vi "editDialog.vi"(0 "reference":refnum<class "StateTransitionEdge.lvclass">, 5 "error in (no error)":errorcluster) -> (14 "reference out":refnum<class "StateTransitionEdge.lvclass">, 15 "cancel":bool, 19 "error out":errorcluster)   [LabVIEW 2020, in "StateTransitionEdge.lvclass"]
doc: "Edit Dialog"
uses:
  <resource>/Framework/Providers/Open_GDS/UML/StateTransitionEdge_class/StateTransitionEdge.lvclass
  C:/Program Files (x86)/National Instruments/LabVIEW 2020/resource/Framework/Providers/Open_GDS/UML/ClassRelationshipEdge_class/ClassRelationshipEdge.lvclass
  C:/Program Files (x86)/National Instruments/LabVIEW 2020/resource/Framework/Providers/Open_GDS/UML/SegmentedLineEdge_class/SegmentedLineEdge.lvclass
  <resource>/Framework/Providers/Open_GDS/UML/BentStyle_class/BentStyleType.ctl
  <resource>/Framework/Providers/Open_GDS/UML/ContextHelp/ContextHelp_HelpTexts.ctl
  <resource>/Framework/Providers/Open_GDS/UML/BentStyle_class/BentStyle.lvclass
  <resource>/Framework/Providers/Open_GDS/UML/ClassRelationshipEdge_class/ClassRelationshipEdge.lvclass
  <resource>/Framework/Providers/Open_GDS/UML/SegmentedLineEdge_class/SegmentedLineEdge.lvclass
panel:
  in  "Bent Style":T1
  in  "Help":bool
  in  "Event":string
  in  "Cancel Button":bool
  in  "OK Button":bool
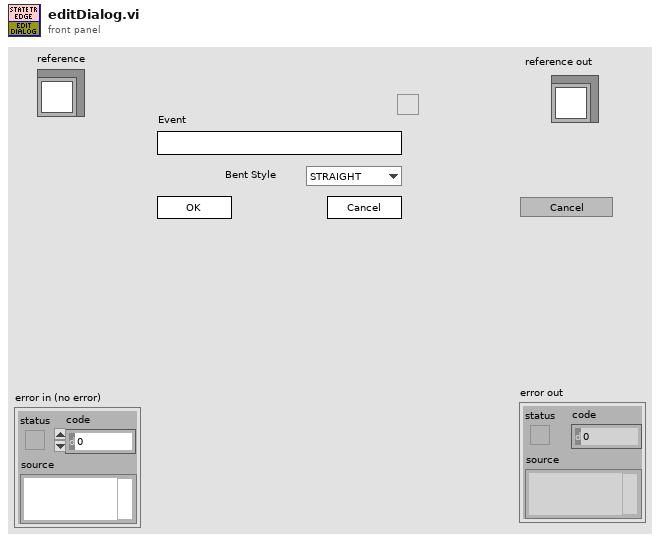
[diagram p1: front panel]
types:
  T1 = typedef "BentStyle.lvclass/BentStyleType.ctl" = enum16{"STRAIGHT", "HV", "VH", "HVH", "VHV", "ARC"}
  T2 = typedef "ContextHelp_HelpTexts.ctl" = enum16{"None(Hide)", "Default", "Help", "Welcome", "GettingStarted", "ClassDiagram_Help", "SequenceDiagram_Help", "UseCaseDiagram_Help", "BSelect", "BClass", "BInterface", "BPackage", "BNote", "BDependency", "BInheritance", "BInterfaceImplementation", "BAssociation", "BAggregation", "BCompAggregation", "BNoteConnector", "BObject", "BActionBar", "BCall", "BSystem", "BActor", "BUseCase", "BGeneralization", "BIncludes", "BExtends", "BUseCaseDiagramAssociation", "ClassRelationshipEdge editDialog_Bent Style", "ClassRelationshipEdge editDialog_RelationType", "ClassRelationshipEdge editDialog_Reverse association", "ClassRelationshipEdge editDialog_Start label", "ClassRelationshipEdge editDialog_Middle label", "ClassRelationshipEdge editDialog_End label", "UMLEditor reversedEngineering_Pathes", "ReversedEngineering StateReverseDialog_Help", "ReversedEngineering StateQueuedSettings_Help", "UMLEditor reversedEngineering_AddTopVIs", "UMLEditor reversedEngineering_AddClasses", "UMLEditor reversedEngineering_AddDirs", "UMLEditor reversedEngineering_Recursively", "UMLEditor reversedEngineering_Remove", "UMLEditor reversedEngineering_ClearList", "UMLEditor reversedEngineering_HideSubAss", "UMLEditor reversedEngineering_CreateTypes", "UMLEditor reversedEngineering_OnlyInheritance", "UMLEditor reversedEngineering_CreateApplication", "UMLEditor reversedEngineering_OK", "UMLEditor reversedEngineering_Cancel", "UMLEditor reversedEngineering_Help", "UMLEditor createWizardScriptFile_ScriptfilePath", "UMLEditor createWizardScriptFile_ClassPath", "UMLEditor createWizardScriptFile_Use", "UMLEditor createWizardScriptFile_PrivateDirName", "UMLEditor createWizardScriptFile_DirAppend", "UMLEditor createWizardScriptFile_Separator Character", "UMLEditor createWizardScriptFile_OK", "UMLEditor createWizardScriptFile_Cancel", "UMLEditor createWizardScriptFile_Help", "ClassNode editDialog_Class Name", "InterfaceNode editDialog_Class Name", "ClassNode editDialog_Attribute", "ClassNode editDialog_Methods", "InterfaceNode editDialog_Methods", "ClassNode editDialog_connection", "InterfaceNode editDialog_connection", "ClassNode editDialog_StereoType", "ClassNode editDialog_ShowAttrib", "ClassNode editDialog_ShowMethods", "ClassNode editDialog_ClassPath", "ClassNode editDialog_AddAttribute", "ClassNode editDialog_AddMethod", "InterfaceNode editDialog_AddMethod", "ClassNode AttributeGuide_AttributeName", "ClassNode AttributeGuide_Array?", "ClassNode AttributeGuide_Data Type", "ClassNode AttributeGuide_RefName", "ClassNode AttributeGuide_Preview", "ClassNode AttributeGuide_OK", "ClassNode AttributeGuide_Cancel", "ClassNode MethodGuide_Visibility", "ClassNode MethodGuide_Method Name", "ClassNode MethodGuide_Preview", "ClassNode MethodGuide_OK", "ClassNode MethodGuide_Cancel", "CallNode EditCallProperties_AllButtons", "ObjectNode EditObjectlProperties_AllButtons", "ActorNode EditActorProperties_AllButtons", "UseCaseRelationshipNode EditUseCaselProperties_AllButtons", "UseCaseNode EditUseCaselProperties_AllButtons", "SystemNode EditSystemProperties_AllButtons", "ReversedEngineering UpdateAttributes_AllButtons", "StateNode editDialog_AllButtons", "StateTransition editDialog_AllButtons", "ArrangeNodes Main_Picture", "ArrangeNodes Main_Zoom", "ArrangeNodes Main_Auto Zoom", "ArrangeNodes Main_shorten", "ArrangeNodes Main_Min Length", "ArrangeNodes Main_Max Length", "ArrangeNodes Main_increase", "ArrangeNodes Main_decrease", "ArrangeNodes Main_Shake", "ArrangeNodes Main", "BState", "BInitialState", "BFinalState", "BStateTransition", "StateDiagram_Help", "StateDiagram_PropertiesAllButtons", "ReversedEngineering StateReverseDialog_ClearStates", "ReversedEngineering StateReverseDialog_UseQueuedStateMachines", "ReversedEngineering StateReverseDialog_QueuedSettings", "ReversedEngineering StateReverseDialog_SearchForVIs", "ReversedEngineering StateReverseDialog_SearchCriteria", "OptionsDialog_ClassBasePath", "OptionsDialog_VIPath", "OptionsDialog_ApplicationPath", "OptionsDialog_WizDir", "OptionsDialog_IniFilePath", "OptionsDialog_DefineColors", "OptionsDialog_Help", "OptionsDialog_CreateTypes", "ClassRelationshipEdge editDialog_SplitWire"}
  T3 = typedef "ClassRelationshipEdge.lvclass/ObjectAttributes.ctl" = cluster{"bentStyleRef":refnum<class "BentStyle.lvclass">, "startConnectionOffset":cluster{"x":i32, "y":i32}, "endConnectionOffset":cluster{"x":i32, "y":i32}, "MidLineOffset":cluster{"x":i32, "y":i32}, "DepClass":T4}
  T4 = typedef "ReversedEngineering_ViDependencyDetailsType.ctl" = cluster{"ThisVIs/Ctls":path[], "Dependent_VIs/Ctls":path[]}
  T5 = typedef "SegmentedLineEdge.lvclass/ObjectAttributes.ctl" = cluster{"lineStyle":refnum<class "LineStyle.lvclass">, "startArrowHead":refnum<class "ArrowHead.lvclass">, "endArrowHead":refnum<class "ArrowHead.lvclass">, "startLabel":string, "midLabel":string, "endLabel":string, "MidLabelOffset":T6, "SplitWire":bool}
  T6 = typedef "Point Point2D.ctl" = cluster{"x":dbl, "y":dbl}
  T7 = typedef "ContextHelp_ShowType.ctl" = cluster{"Header":string, "Picture":picture, "Text":string}
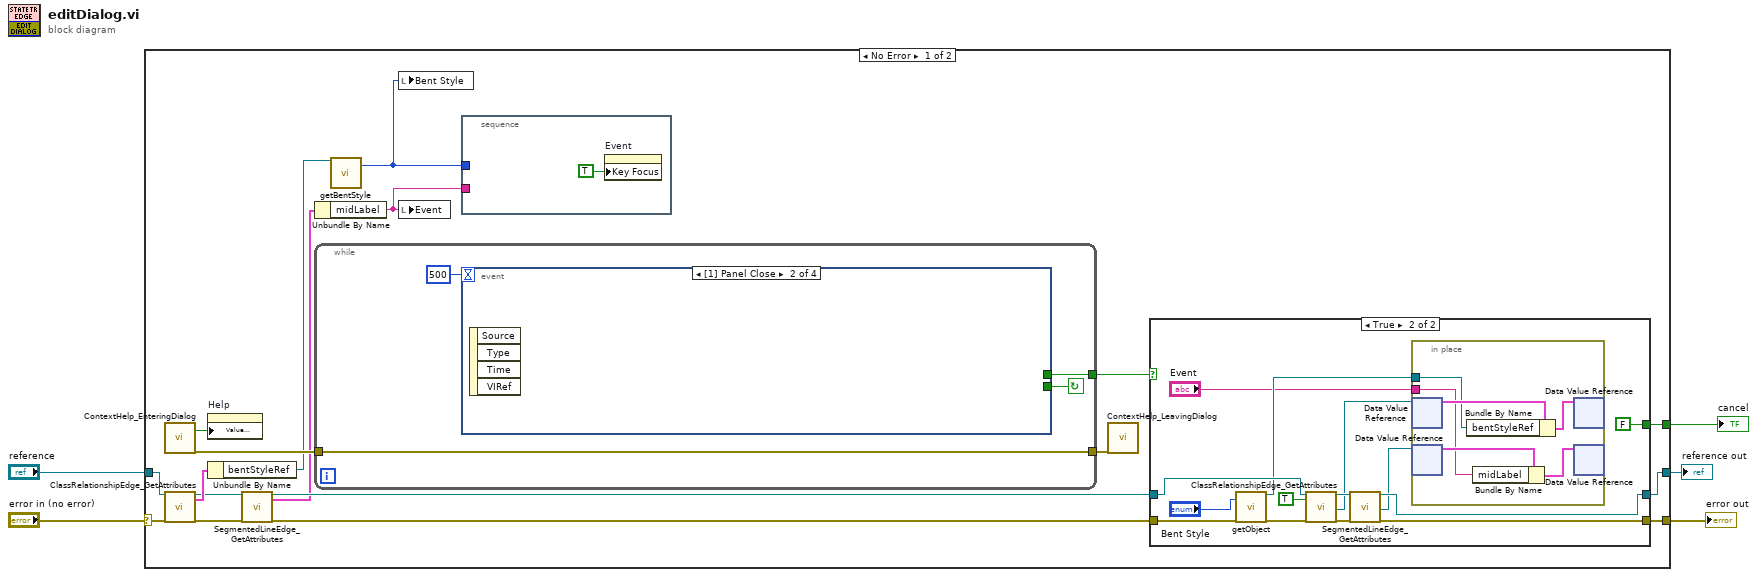
[diagram p0: block diagram]
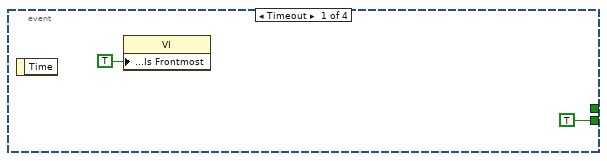
[diagram p2: hidden frame]
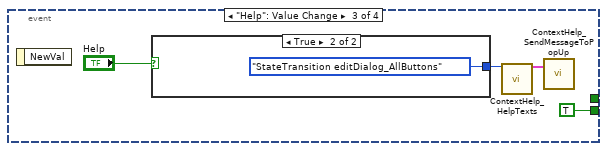
[diagram p3: hidden frame]
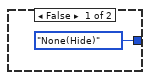
[diagram p4: hidden frame]
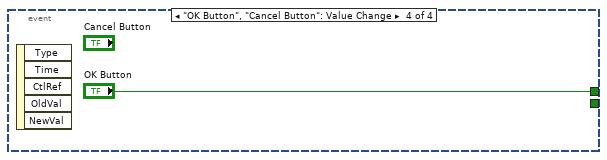
[diagram p5: hidden frame]
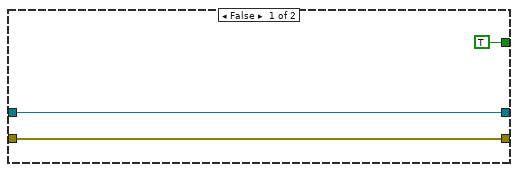
[diagram p6: hidden frame]
diagram:
  n1 = case shown="No Error" "error in (no error)" {
    selector: "error in (no error)" -> [w20 w61]
    tunnel: "reference" -> [w21 w62]
    tunnel: [w23 w61] -> w3
    tunnel: [w22 w62] -> w2
    tunnel: [w17 _] -> w1
    frame No Error {
      n2 = call <resource>:"ContextHelp_EnteringDialog.vi"() -> ("HelpStatus"=w16:bool, "error out"=w14:errorcluster)  [unwired: 3 in, 15 out]
      n3 = call <resource>:"ClassRelationshipEdge_GetAttributes.vi"("reference in"=w21, "error in (no error)"=w20) -> ("reference out"=w10:refnum<class "StateTransitionEdge.lvclass">, "Data"=w11:T3, "error out"=w9:errorcluster)  [unwired: 14 in, 1 out]
      n4 = property on="Help" class="Bool (strict)"("Value (Signaling)"=w16) -> ()  [unwired: 2 in, 2 out]
      n5 = Unbundle By Name(w11) -> ("bentStyleRef"=w13:refnum<class "BentStyle.lvclass">)
      n6 = call <resource>:"SegmentedLineEdge_GetAttributes.vi"("reference in"=w10, "error in (no error)"=w9) -> ("reference out"=w7:refnum<class "StateTransitionEdge.lvclass">, "Data"=w6:T5, "error out"=w8:errorcluster)  [unwired: 14 in, 1 out]
      n7 = Unbundle By Name(w6) -> ("midLabel"=w18:string)
      n8 = while {
        tunnel: [w27] -> w19
        tunnel: [w24] -> w15
        tunnel: w14 -> [w24]
        stop <- w26 continue-if-true
        n9 = event shown="[1] Panel Close" {
          selector: _ -> [_ _ _ _]
          dyn-events: _ -> [_ _ _ _]
          timeout: 500 -> [_ _ _ _]
          tunnel: [_ _ _ "OK Button"] -> w27
          tunnel: [TRUE _ TRUE _] -> w26
          event Timeout {
            n10 = event-data() -> ()  [unwired: 2 out]
            n11 = property class="VI"("Front Panel Window:Is Frontmost"=TRUE) -> ()  [unwired: 2 in, 2 out]
          }
          event Panel Close {
            n12 = event-data() -> ()  [unwired: 5 out]
          }
          event "Help": Value Change {
            n13 = event-data() -> ()  [unwired: 2 out]
            n14 = case shown="True" "Help" {
              tunnel: [ContextHelp_HelpTexts."None(Hide)" ("HelpText") ContextHelp_HelpTexts."StateTransition editDialog_AllButtons" ("HelpText")] -> w32
              frame False {
              }
              frame True {
              }
            }
            n15 = call <resource>:"ContextHelp_HelpTexts.vi"("HelpText (enum or string)"=w32) -> ("HelpOut"=w33:T7)  [unwired: 18 out]
            n16 = call <resource>:"ContextHelp_SendMessageToPopUp.vi"("PopUpMessage"=w33) -> ()  [unwired: 2 in, 17 out]
          }
          event "OK Button", "Cancel Button": Value Change {
            n17 = event-data() -> ()  [unwired: 6 out]
          }
        }
      }
      n18 = call-dynamic "getBentStyle.vi"("reference"=w13) -> ("bentStyle"=w12:T1)  [unwired: 1 in, 17 out]
      n19 = local write "Bent Style"(w12) -> ()
      n20 = local write "Event"(w18) -> ()
      n21 = stacked-sequence {
        tunnel: w18 -> [_]
        tunnel: w12 -> [_]
        frame #0 {
          n22 = property on="Event" class="Str"("Key Focus"=TRUE) -> ()  [unwired: 2 in, 2 out]
        }
      }
      n23 = call <resource>:"ContextHelp_LeavingDialog.vi"("error in (no error)"=w15) -> ()  [unwired: 2 in, 17 out]
      n24 = case shown="True" w19 {
        tunnel: [w37 w53] -> w23
        tunnel: [w39 w52] -> w22
        tunnel: w7 -> [w39 w51]
        tunnel: [TRUE ("Key Focus") FALSE ("Key Focus")] -> w17
        tunnel: w8 -> [w37 w49]
        frame False {
        }
        frame True {
          n25 = call <resource>:"getObject.vi"("bentStyle"="Bent Style", "error in (no error)"=w49) -> ("reference out"=w41:refnum<class "BentStyle.lvclass">, "error out"=w48:errorcluster)  [unwired: 16 out]
          n26 = call <resource>:"ClassRelationshipEdge_GetAttributes.vi"("reference in"=w51, "OnlyGetDvrReference(False)"=TRUE, "error in (no error)"=w48) -> ("reference out"=w45:refnum<class "StateTransitionEdge.lvclass">, "DataRef"=w43:refnum<data-value>, "error out"=w44:errorcluster)  [unwired: 13 in, 1 out]
          n27 = call <resource>:"SegmentedLineEdge_GetAttributes.vi"("reference in"=w45, "error in (no error)"=w44) -> ("reference out"=w52:refnum<class "StateTransitionEdge.lvclass">, "DataRef"=w42:refnum<data-value>, "error out"=w53:errorcluster)  [unwired: 14 in, 1 out]
          n28 = in-place {
            in-place-border: w41 -> [w58]
            in-place-border: "Event" -> [w55]
            n29 = in-place-dvr #1(w43) -> (w59:T3)  [unwired: 1 out]
            n30 = in-place-dvr #2(w42) -> (w56:T5)  [unwired: 1 out]
            n31 = Bundle By Name(cluster=w59, "bentStyleRef"=w58) -> (w57:T3)
            n32 = Bundle By Name(cluster=w56, "midLabel"=w55) -> (w54:T5)
            n33 = in-place-dvr #1(w57) -> ()  [unwired: 2 out]
            n34 = in-place-dvr #2(w54) -> ()  [unwired: 2 out]
          }
        }
      }
    }
    frame Error {
    }
  }
  "reference out" <- w2
  "error out" <- w3
  "cancel" <- w1
